vi "Register Q.vi"(8 "error in (no error)":errorcluster, 9 "Identities":refnum<class "Identity.lvclass">[](array[class]), 10 "MessageQ":refnum<class "MessageQ.lvclass">, 11 "VolatusAPI in":refnum<class "VolatusAPI.lvclass">) -> (0 "error out":errorcluster, 2 "Q Number":i32, 3 "VolatusAPI out":refnum<class "VolatusAPI.lvclass">)   [LabVIEW 2020, in "Volatus.lvlib" / "VolatusAPI.lvclass"]
uses:
  VolatusAPI.lvclass
  MessageQ/MessageQ.lvclass
  Identity/Identity.lvclass
  Q Info.ctl
  VolatusAPI.lvclass/VolatusAPI.ctl
  Registered Q.ctl
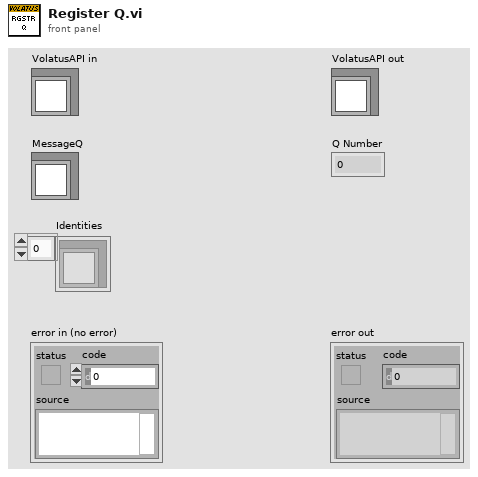
[diagram p1: front panel]
types:
  T1 = typedef "Volatus.lvlib/VolatusAPI.lvclass/Q Info.ctl" = cluster{"Number":i32, "Notifiers":refnum<notifier>[]}
  T2 = typedef "Volatus.lvlib/VolatusAPI.lvclass/Registered Q.ctl" = cluster{"Q":refnum<class "MessageQ.lvclass">, "Keys":string[]}
  T3 = typedef "Volatus.lvlib/VolatusAPI.lvclass/MsgQs Ref.ctl" = cluster{"Keys":map{string, T1}, "MsgQs":map{i32, T2}, "Next Number":i32}
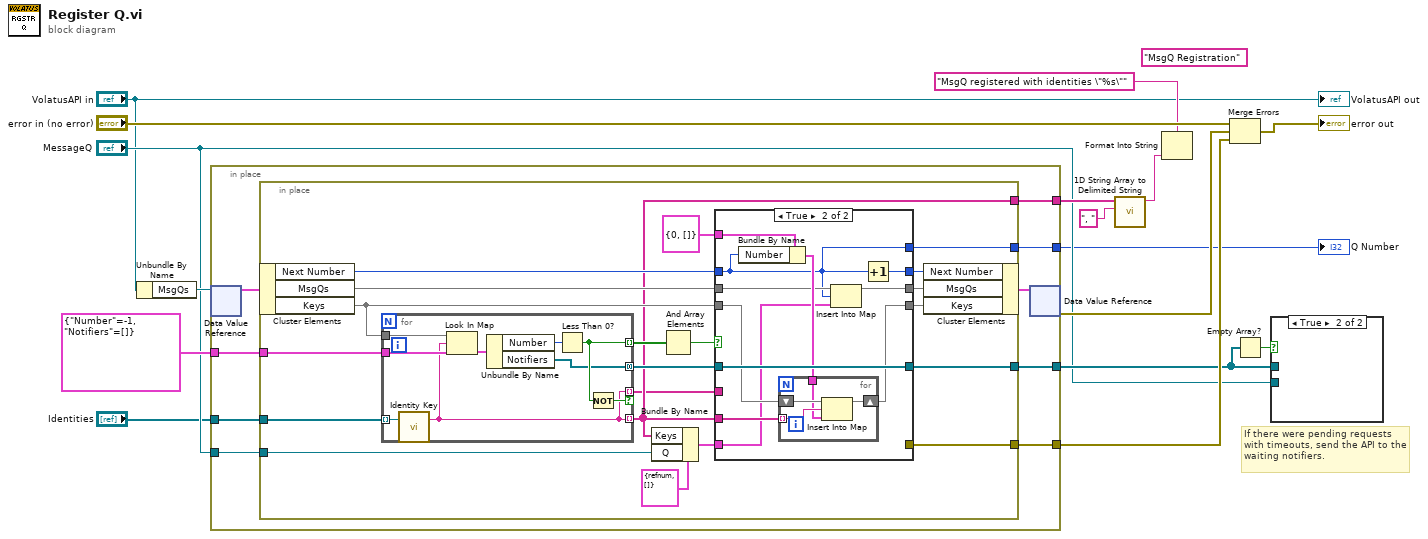
[diagram p0: block diagram]
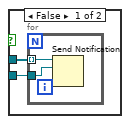
[diagram p2: hidden frame]
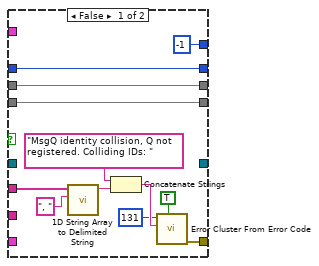
[diagram p3: hidden frame]
diagram:
  (unwired) "MsgQ Registration" ("Context")
  # "If there were pending requests with timeouts, send the API to the waiting notifiers."
  n1 = Unbundle By Name("VolatusAPI in") -> ("MsgQs"=w13:refnum<data-value>)
  n2 = in-place {
    in-place-border: "MessageQ" -> [w24]
    in-place-border: [w23] -> w12
    in-place-border: T1 {"Number"=-1, "Notifiers"=[]} ("default value") -> [w22]
    in-place-border: [w20] -> w6
    in-place-border: [w19] -> w9
    in-place-border: [w18] -> w4
    in-place-border: "Identities" -> [w17]
    n3 = in-place-dvr #1(w13) -> (w25:T3)  [unwired: 1 out]
    n4 = in-place {
      in-place-border: w24 -> [w32]
      in-place-border: [w34] -> w23
      in-place-border: w22 -> [w44]
      in-place-border: [w37] -> w20
      in-place-border: [w28] -> w19
      in-place-border: [w27] -> w18
      in-place-border: w17 -> [w26]
      n5 = in-place-cluster #2(w25) -> ("Next Number"=w39:i32, "MsgQs"=w40:map{i32, T2}, "Keys"=w41:map{string, T1})
      n6 = for {
        tunnel: w26 -> [w54] mode=indexing
        tunnel: w41 -> [w53]
        tunnel: [w49] -> w45 mode=indexing
        tunnel: [w46] -> w34 mode=indexing
        tunnel: [w46] -> w29 mode=indexing if=w48
        tunnel: w44 -> [w52]
        tunnel: [w47] -> w42 mode=concatenating
        n7 = call "Identity Key.vi"("Identity in"=w54) -> ("Identity Key"=w46:string)  [unwired: 2 in]
        n8 = Look In Map(map=w53, key=w46, default value=w52) -> (value=w51:T1)  [unwired: 1 out]
        n9 = Unbundle By Name(w51) -> ("Number"=w50:i32, "Notifiers"=w47:refnum<notifier>[])
        n10 = Less Than 0?(x=w50) -> (x < 0?=w49:bool)
        n11 = Not(x=w49) -> (.not. x?=w48:bool)
      }
      n12 = Bundle By Name(cluster=T2 {"Q"=refnum, "Keys"=[]} ("Registered API"), "Keys"=w34, "Q"=w32) -> (w31:T2)
      n13 = And Array Elements(Boolean array=w45) -> (logical AND=w43:bool)
      n14 = case shown="True" w43 {
        tunnel: w42 -> [_ w76]
        tunnel: w41 -> [w64 w74]
        tunnel: w40 -> [w65 w70]
        tunnel: w39 -> [w66 w67]
        tunnel: [w66 w77] -> w38
        tunnel: [_ w76] -> w37
        tunnel: T1 {"Number"=0, "Notifiers"=[]} ("API Info") -> [_ w75]
        tunnel: [w64 w73] -> w35
        tunnel: w34 -> [_ w71]
        tunnel: w31 -> [_ w68]
        tunnel: [w65 w69] -> w30
        tunnel: w29 -> [w57 _]
        tunnel: [w56 _] -> w28
        tunnel: [-1 ("Next Number") w67] -> w27
        frame False {
          n15 = call <vilib>:"1D String Array to Delimited String.vi"("delimiter"=", ", "string array"=w57) -> ("delimited string"=w62:string)  [unwired: 9 in]
          n16 = Concatenate Strings("MsgQ identity collision, Q not registered. Colliding IDs: ", w62) -> (w63:string)
          n17 = call <vilib>:"Error Cluster From Error Code.vi"("show call chain? (False)"=TRUE, "error message (\"\")"=w63, "error code (0)"=131) -> ("error out"=w56:errorcluster)  [unwired: 6 in]
        }
        frame True {
          n18 = Bundle By Name(cluster=w75, "Number"=w67) -> (w72:T1)
          n19 = for {
            tunnel: w71 -> [w81] mode=indexing
            shift-right: [w79] -> w73
            shift-left: w74 -> [w80]
            tunnel: w72 -> [w78]
            n20 = Insert Into Map(map in=w80, key=w81, value=w78) -> (map out=w79:map{string, T1})  [unwired: 2 out]
          }
          n21 = Insert Into Map(map in=w70, key=w67, value=w68) -> (map out=w69:map{i32, T2})  [unwired: 2 out]
          n22 = Increment(x=w67) -> (x+1=w77:i32)
        }
      }
      n23 = in-place-cluster #2("Next Number"=w38, "MsgQs"=w30, "Keys"=w35) -> (w21:T3)
    }
    n24 = in-place-dvr #1(w21) -> (w8:errorcluster)  [unwired: 1 out]
  }
  "Q Number" <- w4
  n25 = call <vilib>:"1D String Array to Delimited String.vi"("delimiter"=", ", "string array"=w12) -> ("delimited string"=w14:string)  [unwired: 9 in]
  n26 = Format Into String(format string="MsgQ registered with identities \"%s\"", w14) -> ()  [unwired: 2 in, 2 out]
  n27 = Merge Errors("error in (no error)", w8, w9) -> (→"error out":errorcluster)
  n28 = Empty Array?(array=w6) -> (empty?=w7:bool)
  n29 = case shown="True" w7 {
    tunnel: w6 -> [w83 _]
    tunnel: "MessageQ" -> [w82 _]
    frame False {
      n30 = for {
        tunnel: w83 -> [w85] mode=indexing
        tunnel: w82 -> [w84]
        n31 = Send Notification(notification=w84, notifier=w85) -> ()  [unwired: 1 in, 2 out]
      }
    }
    frame True {
    }
  }
  "VolatusAPI out" <- "VolatusAPI in"
